vi "list available jl functions.vi"(8 "error in (no error)":errorcluster) -> (0 "error out":errorcluster, 1 "Jl Server state out":T1, 2 "all_fns":string[](array[string]), 3 "ext_fns":string[](array[string]), 4 "detailed error info":T2, 5 "return code":u8, 7 "timeout?":bool)   [LabVIEW 2018, in "LV2Julia_core.lvlib"]
doc: "List function available on Server."
uses:
  LV2Julia_core.lvlib
  detailed error info.ctl
  StackFrame.ctl
  Server or client state.ctl
  318091ce-7b2e-4b52-a944-14c6363efdda.vi
  318091ce-7b2e-4b52-a944-14c6363efdda.vi/2efcc740-86e8-4604-a8c1-dd245ae1632b.vi
  318091ce-7b2e-4b52-a944-14c6363efdda.vi/2efcc740-86e8-4604-a8c1-dd245ae1632b.vi/967f86db-3e49-41f4-979e-b80f4ab6020c.vi
  318091ce-7b2e-4b52-a944-14c6363efdda.vi/2efcc740-86e8-4604-a8c1-dd245ae1632b.vi/2938b923-4031-45f9-af0f-e581385c98f2.vi
  318091ce-7b2e-4b52-a944-14c6363efdda.vi/2efcc740-86e8-4604-a8c1-dd245ae1632b.vi/158c2851-8195-43bc-815b-080707f0b898.vi
  check ID validity.vi
  bindata_descr to JSON.vi
  check cluster field names.vi
  concat JSON.vi
  build request.vi
  REQ full lifecycle.vi
  Parse server response.vi
  log jl exceptions.vi
panel:
  out "JSON received":string
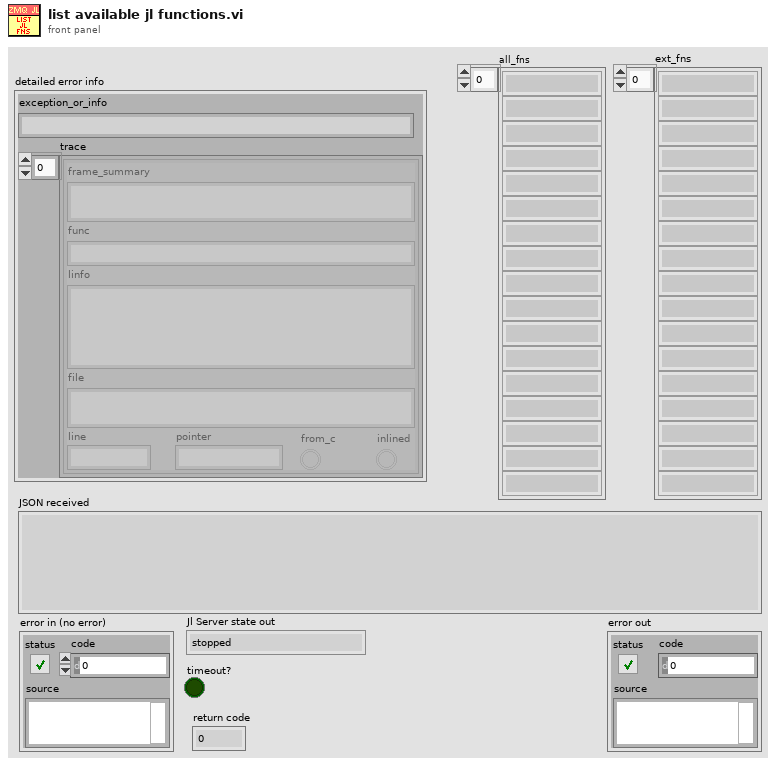
[diagram p1: front panel]
types:
  T1 = typedef "LV2Julia_core.lvlib/Server or client state.ctl" = enum16{"stopped", "running", "unknown"}
  T2 = typedef "LV2Julia_core.lvlib/detailed error info.ctl" = cluster{"exception_or_info":string, "trace":T3[]}
  T3 = typedef "LV2Julia_core.lvlib/StackFrame.ctl" = cluster{"frame_summary":string, "func":string, "linfo":string, "file":string, "line":i32, "pointer":u64, "from_c":bool, "inlined":bool}
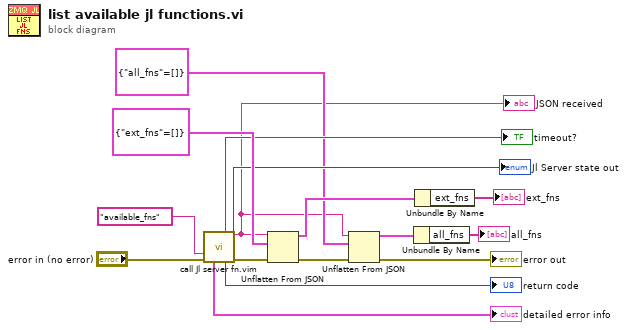
[diagram p0: block diagram]
diagram:
  n1 = call "call Jl server fn.vim"("fun2call"="available_fns", "error in (no error)"="error in (no error)") -> ("timeout?"=→"timeout?":bool, "JSON received"=w4:string, "Jl Server state out"=→"Jl Server state out":T1, "detailed error info"=→"detailed error info":T2, "return code"=→"return code":u8, "error out"=w8:errorcluster)  [unwired: 7 in, 1 out]
  "JSON received" <- w4
  n2 = Unflatten From JSON(JSON string=w4, type and defaults=cluster{"ext_fns":string[]} {"ext_fns"=[]}, error in (no error)=w8) -> (value=w15:cluster{"ext_fns":string[]}, error out=w6:errorcluster)  [unwired: 4 in]
  n3 = Unflatten From JSON(JSON string=w4, type and defaults=cluster{"all_fns":string[]} {"all_fns"=[]}, error in (no error)=w6) -> (value=w3:cluster{"all_fns":string[]}, error out=→"error out":errorcluster)  [unwired: 4 in]
  n4 = Unbundle By Name(w3) -> ("all_fns"=→"all_fns":string[])
  n5 = Unbundle By Name(w15) -> ("ext_fns"=→"ext_fns":string[])
